vi "Plugin_Start.vi"(8 "error in (no error)":errorcluster={"status"=FALSE, "code"=0, "source"="\"\""}, 10 "typed args":string, 11 "Plugin ID":string) -> (0 "error out":errorcluster={"status"=FALSE, "code"=0, "source"="\"\""}, 2 "status ok":bool, 3 "Instance ID":string)   [LabVIEW 2026]
doc: "INTENT: Launch registered plugin worker. LOGIC: Allocate predeployed worker slot; start asynchronously or enqueue to prestarted worker; return immediately."
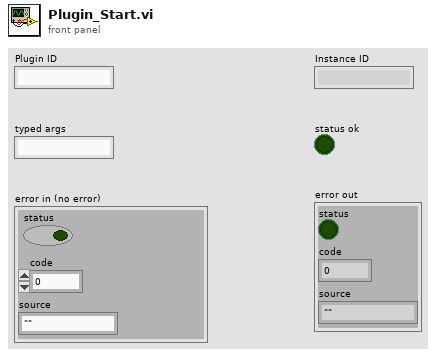
[diagram p1: front panel]
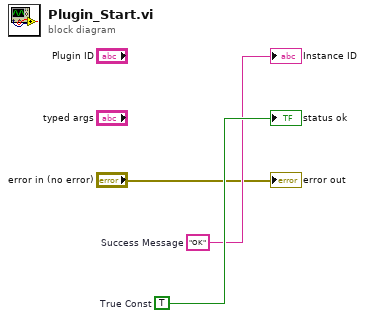
[diagram p0: block diagram]
diagram:
  w3 = TRUE  # True Const
  w2 = "OK"  # Success Message
  "Instance ID" <- w2
  "status ok" <- w3
  "error out" <- "error in (no error)"
